vi "save Screenshot File.vi"(8 "error in (no error)":errorcluster, 10 "File Path":path, 11 "Keysight 9020A in":refnum<class "Keysight 9020A.lvclass">) -> (0 "error out":errorcluster, 3 "Keysight 9020A out":refnum<class "Keysight 9020A.lvclass">)   [LabVIEW 2023, in "Spectrum Analyzer.lvlib" / "Keysight 9020A.lvclass"]
uses:
  Keysight 9020A.lvclass
  Keysight 9020A.lvclass/Keysight 9020A.ctl
  Spectrum Analyzer.lvlib
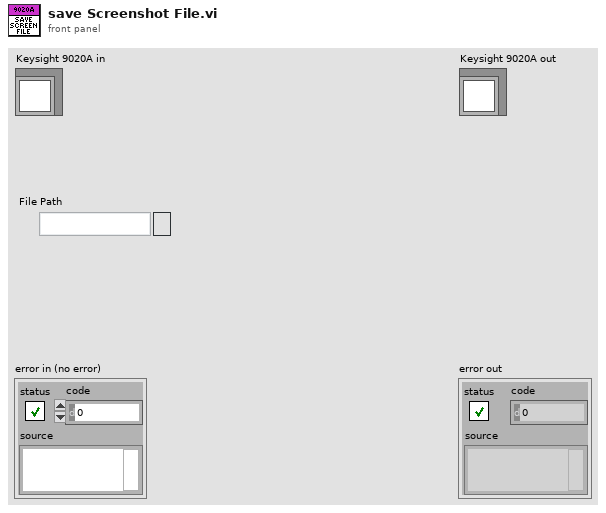
[diagram p1: front panel]
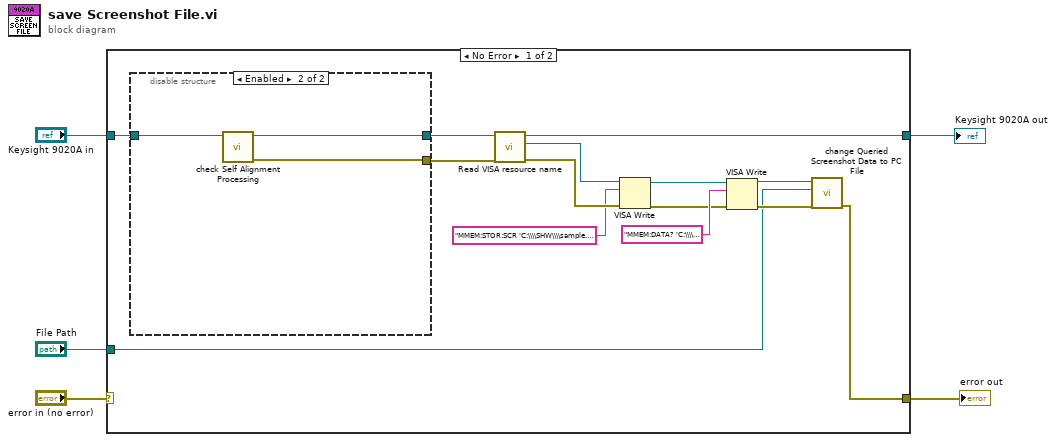
[diagram p0: block diagram]
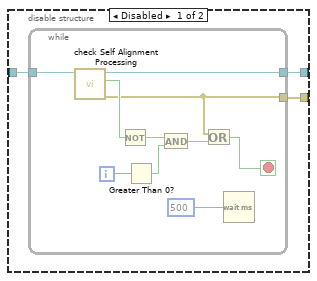
[diagram p2: hidden frame]
diagram:
  n1 = case shown="No Error" "error in (no error)" {
    selector: "error in (no error)" -> [_ w36]
    tunnel: "Keysight 9020A in" -> [w17 w37]
    tunnel: [w19 w37] -> w4
    tunnel: [w6 w36] -> w2
    tunnel: "File Path" -> [w7 _]
    frame No Error {
      n2 = disable-structure shown="Enabled" {
        disable-tunnel: w17 -> [w22 w35]
        disable-tunnel: [w21 w34] -> w16
        disable-tunnel: [w20 w33] -> w15
        frame Disabled {
          n3 = while {
            tunnel: w22 -> [w32]
            tunnel: [w26] -> w20
            tunnel: [w24] -> w21
            i -> [w29]
            stop <- w25 stop-if-true
            n4 = call "check Self Alignment Processing.vi"("Keysight 9020A in"=w32) -> ("error out"=w26:errorcluster, "On Alignment Processing"=w31:bool, "Keysight 9020A out"=w24:refnum<class "Keysight 9020A.lvclass">)  [unwired: 8 in]
            n5 = Not(x=w31) -> (.not. x?=w30:bool)
            n6 = Greater Than 0?(x=w29) -> (x > 0?=w28:bool)
            n7 = And(x=w30, y=w28) -> (x .and. y?=w27:bool)
            n8 = Or(x=w26, y=w27) -> (x .or. y?=w25:bool)
            n9 = Wait (ms)(milliseconds to wait=u32 500) -> ()  [unwired: 1 out]
          }
        }
        frame Enabled {
          n10 = call "check Self Alignment Processing.vi"("Keysight 9020A in"=w35) -> ("error out"=w33:errorcluster, "Keysight 9020A out"=w34:refnum<class "Keysight 9020A.lvclass">)  [unwired: 8 in, 1 out]
        }
      }
      n11 = call "Read VISA resource name.vi"("error in (no error)"=w15, "Keysight 9020A in"=w16) -> ("error out"=w14:errorcluster, "VISA resource name"=w18:refnum<visa-resource-name>, "Keysight 9020A out"=w19:refnum<class "Keysight 9020A.lvclass">)  [unwired: 7 in]
      n12 = VISA Write(VISA resource name=w18, write buffer="MMEM:STOR:SCR 'C:\\\\SHW\\\\sample.png';*OPC", error in (no error)=w14) -> (VISA resource name out=w11:refnum<visa-resource-name>, error out=w10:errorcluster)  [unwired: 1 out]
      n13 = VISA Write(VISA resource name=w11, write buffer="MMEM:DATA? 'C:\\\\SHW\\\\sample.png'", error in (no error)=w10) -> (VISA resource name out=w9:refnum<visa-resource-name>, error out=w8:errorcluster)  [unwired: 1 out]
      n14 = call "change Queried Screenshot Data to PC File.vi"("error in"=w8, "File Path"=w7, "VISA resource name In"=w9) -> ("error out"=w6:errorcluster)  [unwired: 7 in, 1 out]
    }
    frame Error {
    }
  }
  "error out" <- w2
  "Keysight 9020A out" <- w4
